vi "Count Logger States.vi"(8 "error in (no error)":errorcluster, 11 "Log Manager Module in":refnum<class "Log Manager Module.lvclass">) -> (0 "error out":errorcluster, 1 "Logger State Counts":map{T1, i32}(c390), 2 "Logger Count":i32, 3 "Log Manager Module out":refnum<class "Log Manager Module.lvclass">)   [LabVIEW 2020, in "VolatusData.lvlib" / "Log Manager Module.lvclass"]
uses:
  Log Manager Module.lvclass
  Log Manager Module.lvclass/Log Manager Module.ctl
  <vilib>/Utility/miscctls.llb/LVMapReplaceAction.ctl
  Logger State.ctl
  VolatusData.lvlib
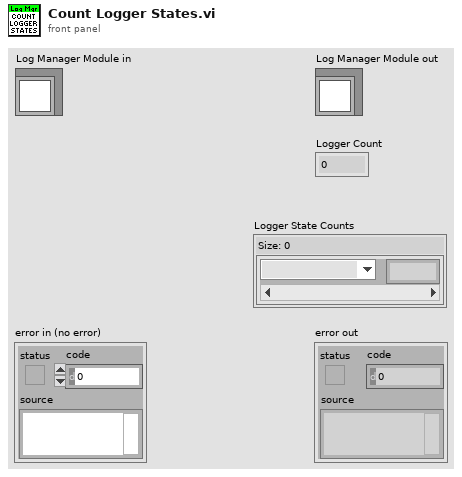
[diagram p1: front panel]
types:
  T1 = typedef "VolatusData.lvlib/Logger State.ctl" = enum16{"Unknown", "Idle", "Preparing", "Ready", "Logging", "Stopping"}
  T2 = typedef "VolatusData.lvlib/Log Manager Module.lvclass/Group Info.ctl" = cluster{"Name":string, "Loggers":map{string, T3}}
  T3 = typedef "VolatusData.lvlib/Log Manager Module.lvclass/Logger.ctl" = cluster{"ID":string, "MsgQ":refnum<class "MessageQ.lvclass">, "State":T1, "Group":string}
  T4 = typedef "LVMapReplaceAction.ctl" = enum32{"Modify Entry only if found", "Add or Modify Entry", "Delete Entry"}
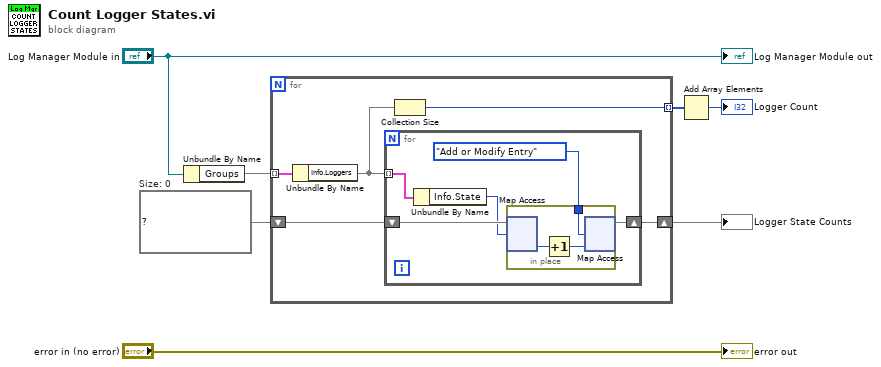
[diagram p0: block diagram]
diagram:
  w6 = map{T1, i32} {}  # Size: 0
  n1 = Unbundle By Name("Log Manager Module in") -> ("Groups"=w5:map{string, T2})
  n2 = for {
    tunnel: w5 -> [w11] mode=indexing
    shift-right: [w10] -> w3
    shift-left: w6 -> [w12]
    tunnel: [w8] -> w2 mode=indexing
    n3 = Unbundle By Name(w11) -> ("Info.Loggers"=w9:map{string, T3})
    n4 = for {
      tunnel: w9 -> [w17] mode=indexing
      shift-right: [w13] -> w10
      shift-left: w12 -> [w16]
      n5 = Unbundle By Name(w17) -> ("Info.State"=w15:T1)
      n6 = in-place {
        in-place-border: LVMapReplaceAction."Add or Modify Entry" ("action") -> [w18]
        n7 = in-place-map #1(w16, w15) -> (w20:i32)  [unwired: 1 in, 1 out]
        n8 = Increment(x=w20) -> (x+1=w19:i32)
        n9 = in-place-map #1(w19, w18) -> (w13:map{T1, i32})  [unwired: 2 out]
      }
    }
    n10 = Collection Size(1:w9) -> (0:w8:i32)
  }
  "Logger State Counts" <- w3
  n11 = Add Array Elements(numeric array=w2) -> (sum=→"Logger Count":i32)
  "error out" <- "error in (no error)"
  "Log Manager Module out" <- "Log Manager Module in"
